vi "Read VI Reference.vi"(8 "error in":errorcluster, 11 "LabVIEW File in":refnum<class "LabVIEW File.lvclass">) -> (0 "error out":errorcluster, 2 "VI Reference":refnum<vi>, 3 "LabVIEW File out":refnum<class "LabVIEW File.lvclass">)   [LabVIEW 2026, in "LabVIEW File.lvclass"]
doc: "Data accessor."
uses:
  LabVIEW File.lvclass
  LabVIEW File.lvclass/LabVIEW File.ctl
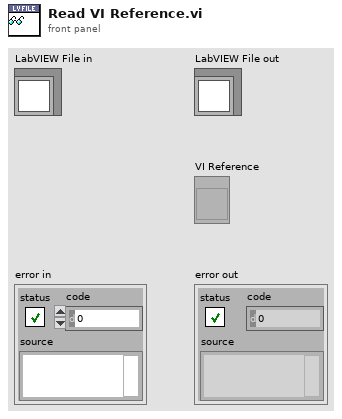
[diagram p1: front panel]
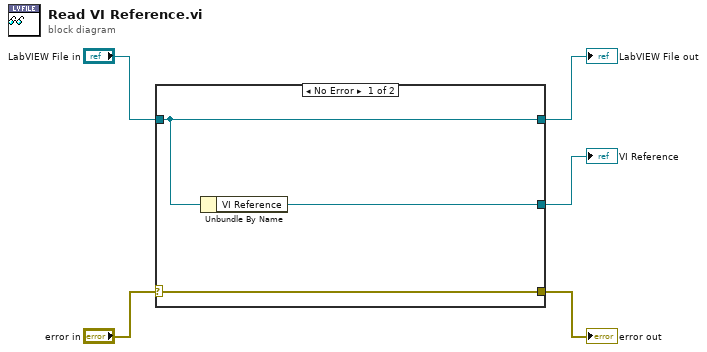
[diagram p0: block diagram]
diagram:
  n1 = case shown="No Error" "error in" {
    selector: "error in" -> [w8 w10]
    tunnel: [w8 w10] -> w4
    tunnel: [w7 w9] -> w2
    tunnel: "LabVIEW File in" -> [w7 w9]
    tunnel: [w6 _] -> w1
    frame No Error {
      n2 = Unbundle By Name(w7) -> ("VI Reference"=w6:refnum<vi>)
    }
    frame Error {
      # "Pass error without further action."
    }
  }
  "error out" <- w4
  "LabVIEW File out" <- w2
  "VI Reference" <- w1
